vi "PicoScope4000aOpen.vi"(0 "USB 3.0 on non-USB 3.0 port control":bool=TRUE, 1 "Serial Number":string, 2 "setProbeInteractionCallback":bool, 3 "Mode":u16(ring) items=["Dialog On Error", "no dialog - CloseUnit and Stop", "no dialog - Continue", "no dialog - Stop"], 5 "Use Serial Number":bool, 7 "Resolution":u32(ring)=1 items=["8-bit", "12-bit", "14-bit"], 9 "USB powered control":bool=TRUE, 11 "error in (no error)":errorcluster) -> (4 "handle":i16, 6 "Pico 4000a Units":string, 8 "count":i16, 10 "Unit Info":T1, 12 "Max ADC value":i16, 13 "USB powered":bool=TRUE, 14 "USB 3.0 on non-USB 3.0 port":bool=TRUE, 15 "error out":errorcluster)   [LabVIEW 2010]
doc: "This VI opens a PicoScope 4000a API device and returns its handle."
uses:
  ps4000aWrap.dll
  ps4000A.dll
panel:
  out "serialLth":i16
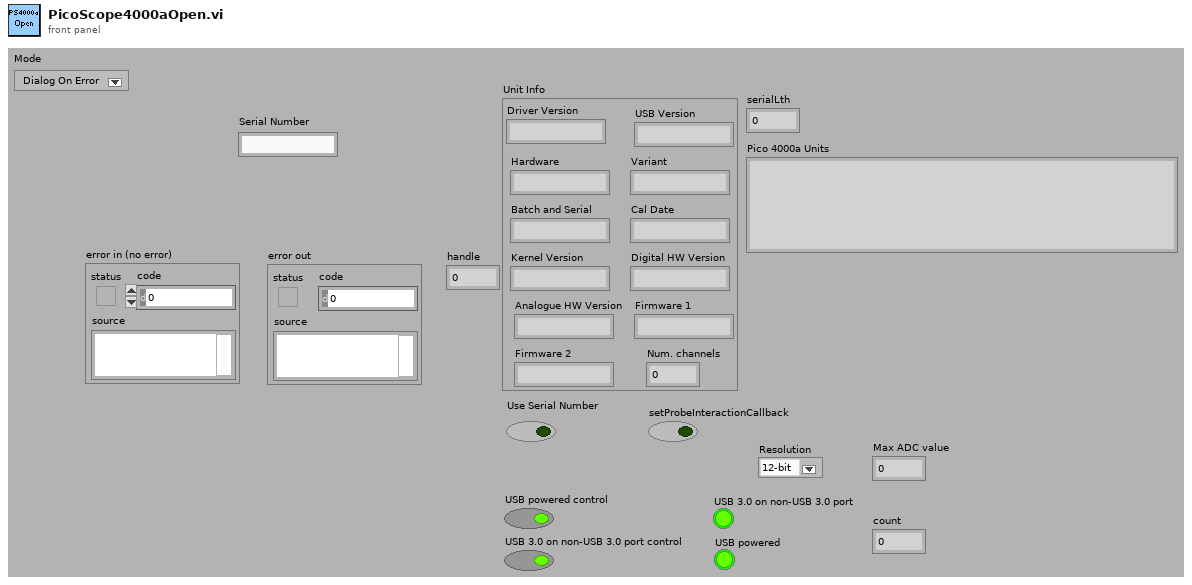
[diagram p1: front panel]
types:
  T1 = cluster{"Driver Version":string, "USB Version":string, "Hardware":string, "Variant":string, "Batch and Serial":string, "Cal Date":string, "Kernel Version":string, "Digital HW Version":string, "Analogue HW Version":string, "Firmware 1":string, "Firmware 2":string, "Num. channels":i16}
  T2 = cluster{"status":bool, "code":u32, "source":string}
  T3 = cluster{"Driver Version":string, "USB Version":string, "Hardware":string, "Variant":string, "Batch and Serial":string, "Cal Date":string, "Kernel Version":string, "Digital HW Version":string, "Analogue HW Version":string, "Firmware 1":string, "Firmware 2":string}
  T4 = cluster{"Driver Version":string, "USB Version":string, "Hardware":string, "Variant":string, "Batch and Serial":string, "Cal Date":string, "Kernel Version":string, "Digital HW Version":string, "Analogue HW Version":string, "Firmware 1":string, "Firmware 2":string, i16}
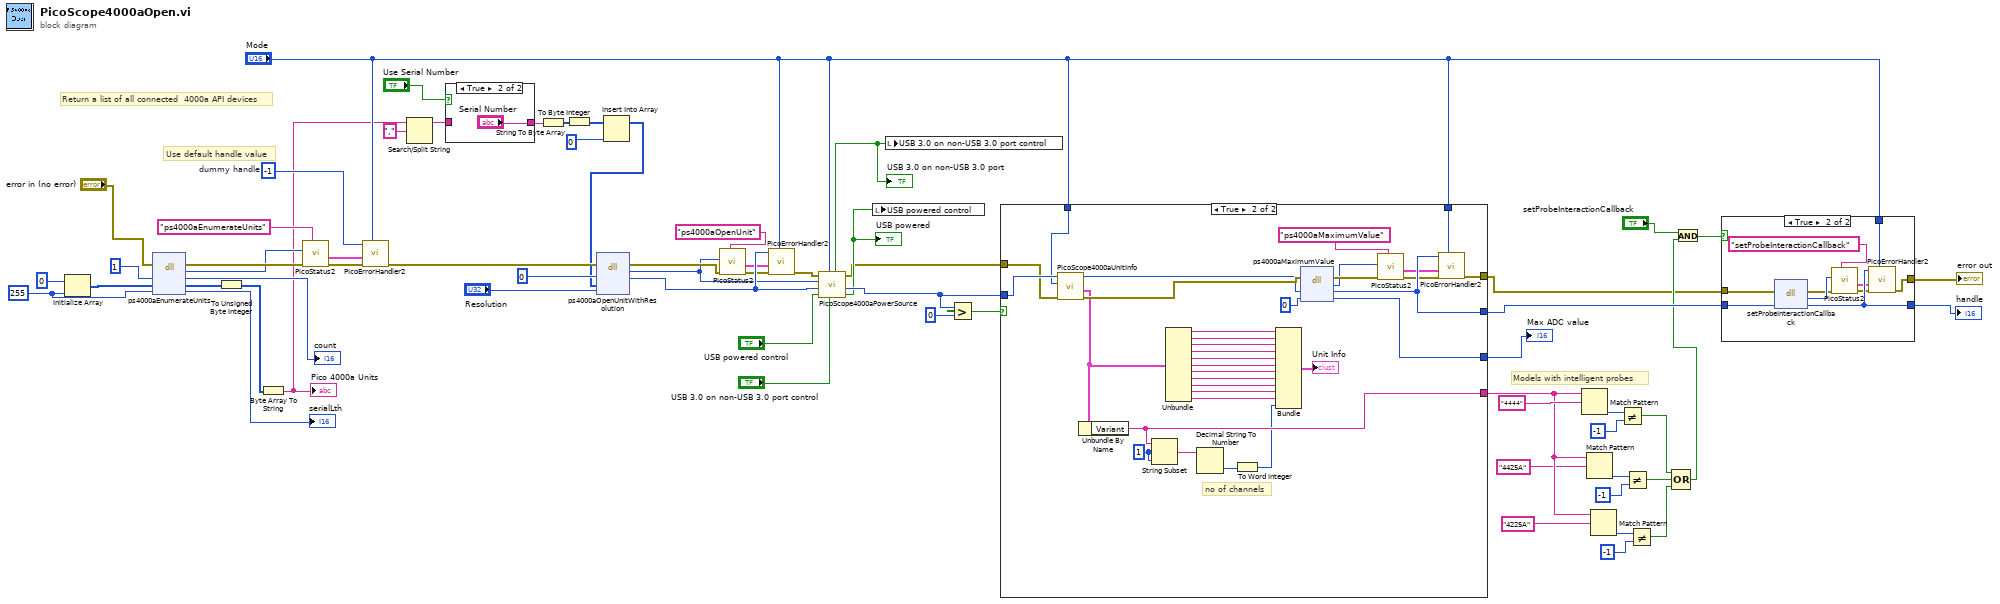
[diagram p0: block diagram]
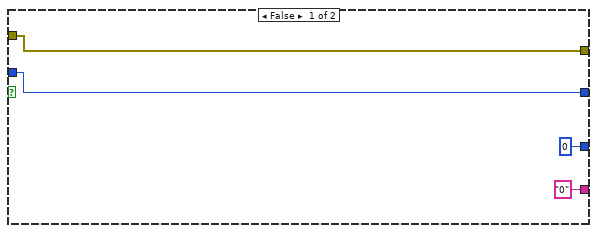
[diagram p4: hidden frame]
diagram:
  w34 = i16 -1  # dummy handle
  w37 = i16 255 ("dimension size")
  # "Models with intelligent probes"
  # "Use default handle value"
  # "Return a list of all connected  4000a API devices"
  n1 = Initialize Array(i8 0 ("U8"), w37) -> (w39:i8[])
  n2 = dll-call lib="ps4000a.dll" fn="ps4000aEnumerateUnits"(error in="error in (no error)", "count"=i16 1, "serials"=w39, "serialLth"=w37) -> (error out=w19:errorcluster, "PICO_STATUS"=w17:u32, "count"=→"count":i16, "serials"=w35:i8[], "serialLth"=→"serialLth":i16)  [unwired: 2 in, 1 out]
  n3 = To Unsigned Byte Integer(number=w35) -> (unsigned 8bit integer=w36:u8[])
  n4 = Byte Array To String(unsigned byte array=w36) -> (string=w8:string)
  "Pico 4000a Units" <- w8
  n5 = call "PicoStatus2.vi"("PICO source"="ps4000aEnumerateUnits" ("source"), "Error in"=w19, "PICO STATUS"=w17) -> ("error out"=w21:errorcluster, "PICO_STATUS out"=w20:T2)  [unwired: 5 in]
  n6 = call "PicoErrorHandler2.vi"("Mode"="Mode", "error in (no error)"=w21, "PICO_STATUS in"=w20, "handle In"=w34) -> ("error out"=w45:errorcluster)  [unwired: 7 in]
  n7 = Search/Split String(string=w8, search string/char (-)=",") -> (substring before match=w6:string)  [unwired: 1 in, 2 out]
  n8 = case shown="True" "Use Serial Number" {
    tunnel: w6 -> [w65 _]
    tunnel: [w65 "Serial Number"] -> w2
    frame False {
    }
    frame True {
    }
  }
  n9 = String To Byte Array(string=w2) -> (unsigned byte array=w4:u8[])
  n10 = To Byte Integer(number=w4) -> (8bit integer=w5:i8[])
  n11 = Insert Into Array(array=w5, new element=i8 0 ("new element/subarray")) -> (w1:i8[])  [unwired: 1 in]
  n12 = dll-call lib="ps4000A.dll" fn="ps4000aOpenUnitWithResolution" ("ps3000.dll:_ps3000_open_unit@0")(error in=w45, "handle"=i16 0, "serial"=w1, "resolution"="Resolution") -> (error out=w14:errorcluster, "PICO_STATUS"=w13:u32, "handle"=w44:i16)  [unwired: 4 in, 1 out]
  n13 = call "PicoStatus2.vi"("PICO source"="ps4000aOpenUnit" ("source"), "Error in"=w14, "PICO STATUS"=w13) -> ("error out"=w12:errorcluster, "PICO_STATUS out"=w16:T2)  [unwired: 5 in]
  n14 = call "PicoErrorHandler2.vi"("Mode"="Mode", "error in (no error)"=w12, "PICO_STATUS in"=w16, "handle In"=w44) -> ("error out"=w57:errorcluster)  [unwired: 7 in]
  n15 = call "PicoScope4000aPowerSource.vi"("USB 3.0 on non-USB 3.0 port control"="USB 3.0 on non-USB 3.0 port control", "Mode"="Mode", "USB powered control"="USB powered control", "handle in"=w44, "PICO STATUS IN"=w13, "error in (no error)"=w57) -> ("USB powered"=w59:bool, "handle out"=w62:i16, "error out"=w56:errorcluster, "USB 3.0 on non-USB 3.0 port"=w58:bool)  [unwired: 1 in, 1 out]
  "USB 3.0 on non-USB 3.0 port" <- w58
  "USB powered" <- w59
  n16 = local write "USB powered control"(w59) -> ()
  n17 = local write "USB 3.0 on non-USB 3.0 port control"(w58) -> ()
  n18 = Greater?(x=w62, y=i16 0) -> (0:w64:bool)
  n19 = case shown="True" w64 {
    tunnel: w62 -> [w70 w103]
    tunnel: [w70 w89] -> w54
    tunnel: w56 -> [w67 w88]
    tunnel: [i16 0 ("value") w87] -> w55
    tunnel: ["0" ("Variant") w85] -> w28
    tunnel: [w67 w75] -> w11
    tunnel: "Mode" -> [_ w74]
    tunnel: "Mode" -> [_ w71]
    frame False {
    }
    frame True {
      w102 = 1 ("offset (0)")
      # "no of channels"
      n20 = call "PicoScope4000aUnitInfo.vi"("error in (no error)"=w88, "Mode"=w71, "handle in"=w103) -> ("error out"=w78:errorcluster, "Unit Info"=w72:T3, "handle out"=w73:i16)  [unwired: 3 in, 1 out]
      n21 = Unbundle By Name(w72) -> ("Variant"=w85:string)
      n22 = String Subset(string=w85, offset (0)=w102, length (rest)=w102) -> (substring=w84:string)
      n23 = Unbundle(w72) -> ("Driver Version"=w101:string, "USB Version"=w100:string, "Hardware"=w99:string, "Variant"=w98:string, "Batch and Serial"=w97:string, "Cal Date"=w96:string, "Kernel Version"=w95:string, "Digital HW Version"=w94:string, "Analogue HW Version"=w93:string, "Firmware 1"=w92:string, "Firmware 2"=w91:string)
      n24 = Decimal String To Number(string=w84) -> (number=w83:i32)  [unwired: 2 in, 1 out]
      n25 = To Word Integer(number=w83) -> (16bit integer=w82:i16)
      n26 = Bundle("Driver Version"=w101, "USB Version"=w100, "Hardware"=w99, "Variant"=w98, "Batch and Serial"=w97, "Cal Date"=w96, "Kernel Version"=w95, "Digital HW Version"=w94, "Analogue HW Version"=w93, "Firmware 1"=w92, "Firmware 2"=w91, w82) -> (→"Unit Info":T4)  [unwired: 1 in]
      n27 = dll-call lib="ps4000a.dll" fn="ps4000aMaximumValue"(error in=w78, "handle"=w73, "value"=i16 0) -> (error out=w81:errorcluster, "PICO_STATUS"=w80:u32, "handle"=w89:i16, "value"=w87:i16)  [unwired: 2 in, 1 out]
      n28 = call "PicoStatus2.vi"("PICO source"="ps4000aMaximumValue" ("source"), "Error in"=w81, "PICO STATUS"=w80) -> ("error out"=w77:errorcluster, "PICO_STATUS out"=w76:T2)  [unwired: 5 in]
      n29 = call "PicoErrorHandler2.vi"("Mode"=w74, "error in (no error)"=w77, "PICO_STATUS in"=w76, "handle In"=w89) -> ("error out"=w75:errorcluster)  [unwired: 7 in]
    }
  }
  "Max ADC value" <- w55
  n30 = Match Pattern(string=w28, regular expression="4444") -> (offset past match=w50:i32)  [unwired: 1 in, 3 out]
  n31 = Match Pattern(string=w28, regular expression="4425A") -> (offset past match=w32:i32)  [unwired: 1 in, 3 out]
  n32 = Match Pattern(string=w28, regular expression="4225A") -> (offset past match=w30:i32)  [unwired: 1 in, 3 out]
  n33 = Not Equal?(x=w50, y=-1) -> (x != y?=w23:bool)
  n34 = Not Equal?(x=w32, y=-1) -> (x != y?=w24:bool)
  n35 = Not Equal?(x=w30, y=-1) -> (x != y?=w25:bool)
  n36 = Compound Arithmetic op=OR(w23, w24, w25) -> (w22:bool)
  n37 = And(x="setProbeInteractionCallback", y=w22) -> (x .and. y?=w48:bool)
  n38 = case shown="True" w48 {
    tunnel: w11 -> [w105 w115]
    tunnel: [w105 w113] -> w53
    tunnel: [w104 w112] -> w52
    tunnel: w54 -> [w104 w114]
    tunnel: "Mode" -> [_ w106]
    frame False {
    }
    frame True {
      n39 = dll-call lib="ps4000aWrap.dll" fn="setProbeInteractionCallback"(error in=w115, "handle"=w114) -> (error out=w107:errorcluster, "PICO_STATUS"=w108:u32, "handle"=w112:i16)  [unwired: 2 in, 1 out]
      n40 = call "PicoStatus2.vi"("PICO source"="setProbeInteractionCallback" ("source"), "Error in"=w107, "PICO STATUS"=w108) -> ("error out"=w111:errorcluster, "PICO_STATUS out"=w110:T2)  [unwired: 5 in]
      n41 = call "PicoErrorHandler2.vi"("Mode"=w106, "error in (no error)"=w111, "PICO_STATUS in"=w110, "handle In"=w112) -> ("error out"=w113:errorcluster)  [unwired: 7 in]
    }
  }
  "handle" <- w52
  "error out" <- w53
